vi "contains.vi"(0 "reference":refnum<class "GeneralPathEdge.lvclass">, 1 "point2D":T1 {"y" format="%.2f"; "x" format="%.2f"}, 2 "GraphicsRef":refnum<class "Graphics.lvclass">, 5 "error in (no error)":errorcluster, 7 "DistanceAwayOffset(100%)":i32=100) -> (14 "reference out":refnum<class "GeneralPathEdge.lvclass">, 15 "contains":bool, 19 "error out":errorcluster)   [LabVIEW 2020, in "GeneralPathEdge.lvclass"]
doc: "public boolean contains(Point2D aPoint)\n {\n final double MAX_DIST = 3;\n\n // the end points may contain small nodes, so don't\n // match them\n Line2D conn = getConnectionPoints();\n if (aPoint.distance(conn.getP1()) <= MAX_DIST \n || aPoint.distance(conn.getP2()) <= MAX_DIST)\n return false;\n\n GeneralPath p = getPath();\n BasicStroke fatStroke = new BasicStroke(\n (float)(2 * MAX_DIST));\n Shape fatPath = fatStroke.createStrokedShape(p);\n return fatPath.contains(aPoint);\n }"
uses:
  <resource>/Framework/Providers/Open_GDS/UML/GeneralPathEdge_class/GeneralPathEdge.lvclass
  C:/Program Files (x86)/National Instruments/LabVIEW 2020/resource/Framework/Providers/Open_GDS/UML/AbstractEdge_class/AbstractEdge.lvclass
  <resource>/Framework/Providers/Open_GDS/UML/General/Point/Point Point2D.ctl
  <resource>/Framework/Providers/Open_GDS/UML/Graphics_class/Graphics.lvclass
  <resource>/Framework/Providers/Open_GDS/UML/AbstractEdge_class/AbstractEdge.lvclass
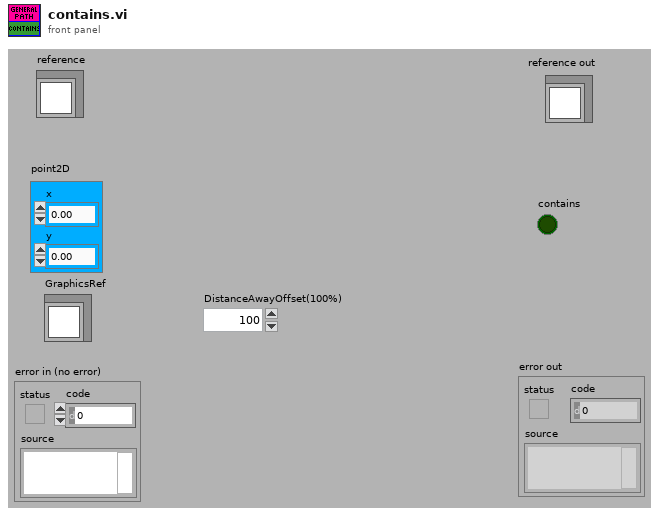
[diagram p1: front panel]
types:
  T1 = typedef "Point Point2D.ctl" = cluster{"x":dbl, "y":dbl}
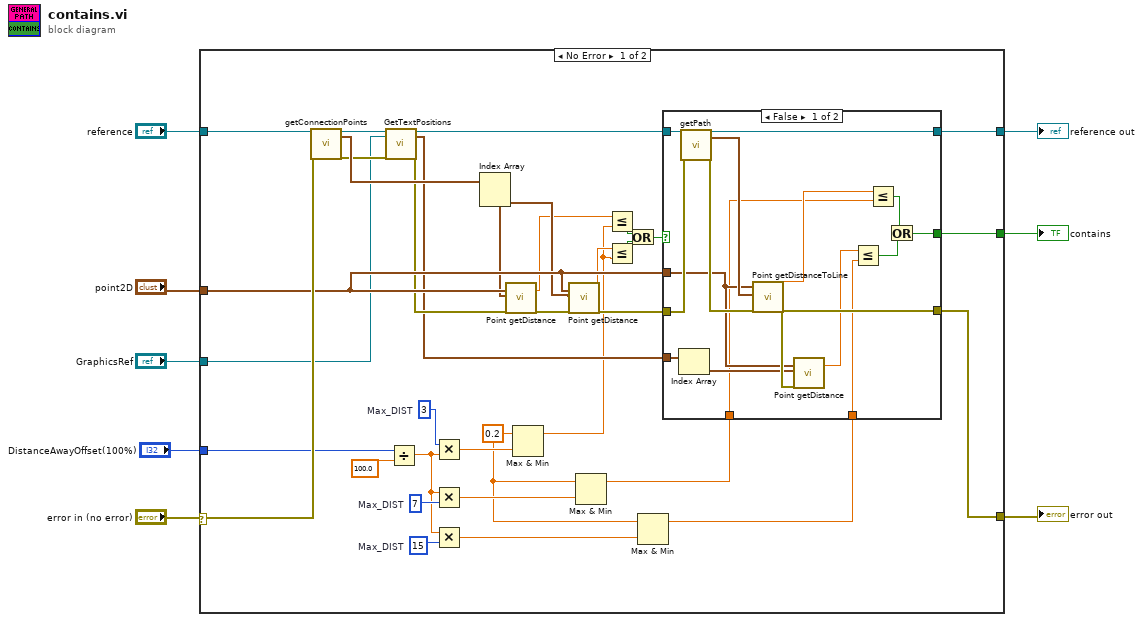
[diagram p0: block diagram]
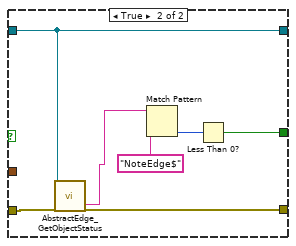
[diagram p2: hidden frame]
diagram:
  n1 = case shown="No Error" "error in (no error)" {
    selector: "error in (no error)" -> [w40 w67]
    tunnel: "reference" -> [w43 w68]
    tunnel: [w42 w67] -> w7
    tunnel: [w41 w68] -> w6
    tunnel: [w39 _] -> w4
    tunnel: "point2D" -> [w38 _]
    tunnel: "GraphicsRef" -> [w22 _]
    tunnel: "DistanceAwayOffset(100%)" -> [w21 _]
    frame No Error {
      w9 = 0.2 ("x")
      w14 = 15  # Max_DIST
      w17 = 7  # Max_DIST
      w19 = 3  # Max_DIST
      n2 = call-dynamic "getConnectionPoints.vi"("reference"=w43, "error in (no error)"=w40) -> ("reference out"=w27:refnum<class "GeneralPathEdge.lvclass">, "connectionPoints"=w37:T1[], "error out"=w25:errorcluster)  [unwired: 15 in]
      n3 = call-dynamic "GetTextPositions.vi"("reference"=w27, "GraphicsRef"=w22, "error in (no error)"=w25) -> ("reference out"=w26:refnum<class "GeneralPathEdge.lvclass">, "connectionPoints"=w23:T1[], "error out"=w24:errorcluster)  [unwired: 14 in]
      n4 = Divide(x=w21, y=100.0) -> (x/y=w15:dbl)
      n5 = Multiply(x=w19, y=w15) -> (x*y=w18:dbl)
      n6 = Multiply(x=w15, y=w17) -> (x*y=w16:dbl)
      n7 = Multiply(x=w15, y=w14) -> (x*y=w13:dbl)
      n8 = Index Array(array=w37) -> (element #1=w35:T1, element #2=w34:T1)  [unwired: 2 in]
      n9 = call <resource>:"Point getDistance.vi"("point1"=w38, "point2"=w35, "error in (no error)"=w24) -> ("distance"=w32:dbl, "error out"=w36:errorcluster)  [unwired: 15 out]
      n10 = Max & Min(x=w9, y=w18) -> (max(x,y)=w12:dbl)  [unwired: 1 out]
      n11 = call <resource>:"Point getDistance.vi"("point1"=w38, "point2"=w34, "error in (no error)"=w36) -> ("distance"=w33:dbl, "error out"=w28:errorcluster)  [unwired: 15 out]
      n12 = Max & Min(x=w9, y=w16) -> (max(x,y)=w11:dbl)  [unwired: 1 out]
      n13 = Less Or Equal?(x=w32, y=w12) -> (x <= y?=w31:bool)
      n14 = Less Or Equal?(x=w33, y=w12) -> (x <= y?=w30:bool)
      n15 = Or(x=w31, y=w30) -> (x .or. y?=w29:bool)
      n16 = Max & Min(x=w9, y=w13) -> (max(x,y)=w10:dbl)  [unwired: 1 out]
      n17 = case shown="False" w29 {
        tunnel: [w47 w61] -> w39
        tunnel: w26 -> [w59 w65]
        tunnel: w28 -> [w58 w66]
        tunnel: w38 -> [w52 _]
        tunnel: [w54 w65] -> w41
        tunnel: [w53 w64] -> w42
        tunnel: w23 -> [w51 _]
        tunnel: w11 -> [w45 _]
        tunnel: w10 -> [w44 _]
        frame False {
          n18 = Index Array(array=w51) -> (element=w50:T1)  [unwired: 1 in]
          n19 = call-dynamic "getPath.vi"("reference"=w59, "error in (no error)"=w58) -> ("reference out"=w54:refnum<class "GeneralPathEdge.lvclass">, "points"=w56:T1[], "error out"=w57:errorcluster)  [unwired: 15 in]
          n20 = call <resource>:"Point getDistanceToLine.vi"("point1"=w52, "line"=w56, "error in (no error)"=w57) -> ("minDistance"=w49:dbl, "error out"=w53:errorcluster)  [unwired: 15 out]
          n21 = call <resource>:"Point getDistance.vi"("point1"=w52, "point2"=w50, "error in (no error)"=w53) -> ("distance"=w48:dbl)  [unwired: 16 out]
          n22 = Less Or Equal?(x=w48, y=w44) -> (x <= y?=w46:bool)
          n23 = Less Or Equal?(x=w49, y=w45) -> (x <= y?=w55:bool)
          n24 = Or(x=w55, y=w46) -> (x .or. y?=w47:bool)
        }
        frame True {
          n25 = call <resource>:"AbstractEdge_GetObjectStatus.vi"("reference in"=w65, "error in (no error)"=w66) -> ("Class name"=w60:string, "error out"=w64:errorcluster)  [unwired: 16 out]
          n26 = Match Pattern(string=w60, regular expression="NoteEdge$") -> (offset past match=w62:i32)  [unwired: 4 out]
          n27 = Less Than 0?(x=w62) -> (x < 0?=w61:bool)
        }
      }
    }
    frame Error {
    }
  }
  "reference out" <- w6
  "error out" <- w7
  "contains" <- w4
